vi "Get Relay States.vi"(8 "error in (no error)":errorcluster, 9 "nodePath":string, 10 "NIVS.System Definition Root":refnum<k24>, 11 "WorkspaceManager in":T1) -> (0 "error out":errorcluster, 1 "MUX Name":string, 2 "Relays":T2[](array[typedef]), 3 "WorkspaceManager out":T1)   [LabVIEW 2013]
uses:
  NationalInstruments.VeriStand.SystemStorage
  SubVIs/Relay Data.ctl
  SubVIs/Switch.ctl
  <vilib>/NI Veristand/Execution/Workspace/WorkspaceAPI.ctl
  NationalInstruments.VeriStand.ClientAPI
  NationalInstruments.VeriStand
  <vilib>/NI Veristand/Execution/Workspace/NI VeriStand - Get Single Channel Value.vi
  MUX Custom Device.lvlib
  <vilib>/NI Veristand/Execution/Workspace/NI_VS Workspace ExecutionAPI.lvlib
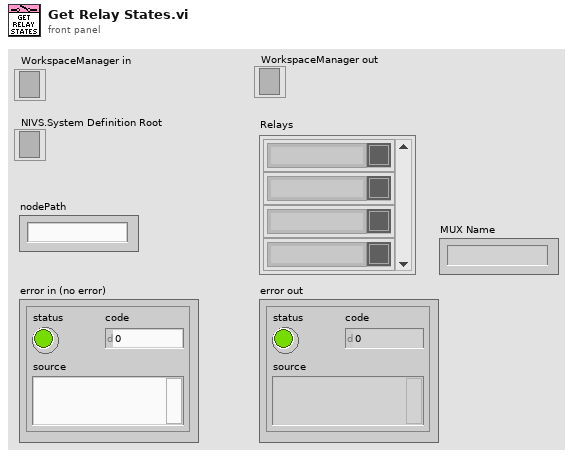
[diagram p1: front panel]
types:
  T1 = typedef "NI_VS Workspace ExecutionAPI.lvlib/WorkspaceAPI.ctl" = refnum<k24>
  T2 = typedef "MUX Custom Device.lvlib/Relay Data.ctl" = cluster{"Relay Name":string, "State":T3}
  T3 = typedef "MUX Custom Device.lvlib/Switch.ctl" = bool
  T4 = typedef "NI_VS Workspace ExecutionAPI.lvlib/SystemState.ctl" = u8
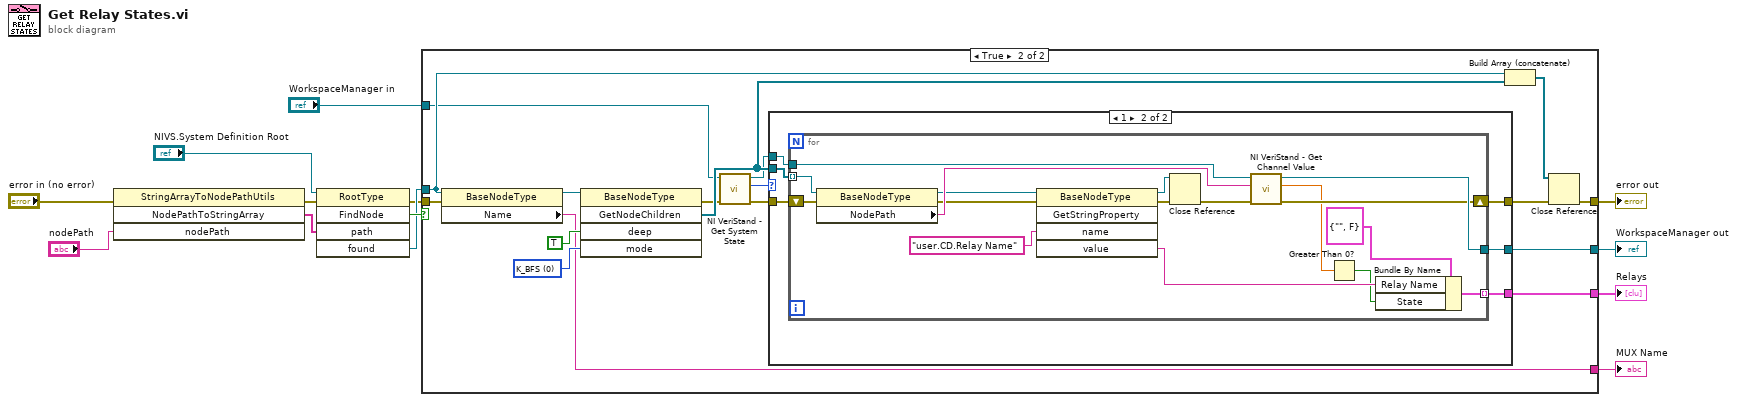
[diagram p0: block diagram]
diagram:
  n1 = invoke class="StringArrayToNodePathUtils" method="NodePathToStringArray"(error in="error in (no error)", "nodePath"="nodePath") -> (error out=w12:errorcluster, "NodePathToStringArray"=w13:string[])  [unwired: 2 in, 2 out]
  n2 = invoke class="RootType" method="FindNode"(reference="NIVS.System Definition Root", error in=w12, "path"=w13) -> (error out=w2:errorcluster, "FindNode"=w9:bool, "found"=w8:refnum<k24>)  [unwired: 2 in, 2 out]
  n3 = case shown="True" w9 {
    tunnel: w2 -> [w15 w24]
    tunnel: w8 -> [_ w23]
    tunnel: "WorkspaceManager in" -> [w14 w18]
    tunnel: [w14 w30] -> w6
    tunnel: [w15 w27] -> w5
    tunnel: [_ w29] -> w4
    tunnel: [_ w21] -> w1
    frame False {
    }
    frame True {
      w31 = 0 items=["K_BFS", "K_DFS", "K_CHILDONLY", "K_UP"] ("mode")
      n4 = property class="BaseNodeType"(reference=w23, error in=w24) -> (reference out=w22:refnum<k24>, "Name"=w21:string)  [unwired: 1 out]
      n5 = invoke class="BaseNodeType" method="GetNodeChildren"(reference=w22, "deep"=TRUE, "mode"=w31) -> (error out=w20:errorcluster, "GetNodeChildren"=w26:refnum<k24>[])  [unwired: 2 in, 3 out]
      n6 = call <vilib>:"NI VeriStand - Get System State.vi"("error in (no error)"=w20, "WorkspaceManager in"=w18) -> ("error out"=w19:errorcluster, "System State"=w16:T4, "WorkspaceManager  out"=w17:T1)  [unwired: 5 in, 2 out]
      n7 = case shown="1" w16 {
        tunnel: [w34 w40] -> w30
        tunnel: [_ w39] -> w29
        tunnel: [w33 w38] -> w28
        tunnel: w26 -> [_ w37]
        tunnel: w19 -> [w33 w36]
        tunnel: w17 -> [w34 w35]
        frame 0, Default {
        }
        frame 1 {
          n8 = for {
            tunnel: w37 -> [w57] mode=indexing
            shift-right: [w54] -> w38
            shift-left: w36 -> [w56]
            tunnel: w35 -> [w44]
            tunnel: [w55] -> w40
            tunnel: [w48] -> w39 mode=indexing
            n9 = property class="BaseNodeType"(reference=w57, error in=w56) -> (reference out=w50:refnum<k24>, error out=w51:errorcluster, "NodePath"=w53:string)
            n10 = invoke class="BaseNodeType" method="GetStringProperty"(reference=w50, error in=w51, "name"="user.CD.Relay Name") -> (reference out=w41:refnum<k24>, error out=w43:errorcluster, "value"=w49:string)  [unwired: 2 in, 2 out]
            n11 = Close Reference(reference=w41, error in (no error)=w43) -> (error out=w42:errorcluster)
            n12 = call-poly <vilib>:"NI VeriStand - Get Channel Value.vi"("error in (no error)"=w42, "Channel"=w53, "WorkspaceManager in"=w44) -> ("error out"=w54:errorcluster, "Value"=w45:dbl, "WorkspaceManager out"=w55:T1)  [unwired: 6 in]
            n13 = Greater Than 0?(x=w45) -> (x > 0?=w47:bool)
            n14 = Bundle By Name(cluster=T2 {"Relay Name"="", "State"=FALSE} ("Relay Data"), "Relay Name"=w49, "State"=w47) -> (w48:T2)
          }
        }
      }
      n15 = Build Array (concatenate)(w23, w26) -> (w25:refnum<k24>[])
      n16 = Close Reference(reference=w25, error in (no error)=w28) -> (error out=w27:errorcluster)
    }
  }
  "Relays" <- w4
  "WorkspaceManager out" <- w6
  "error out" <- w5
  "MUX Name" <- w1
